vi "BUILD_install for dependencies core.vi"(6 "buildlog":path, 8 "error in":errorcluster, 9 "args":string[](array[string]), 11 "vipb path":path) -> (0 "error out":errorcluster)   [LabVIEW 2010]
uses:
  <vilib>/JKI/VIPM API/VIPM API_vipm_api.lvlib
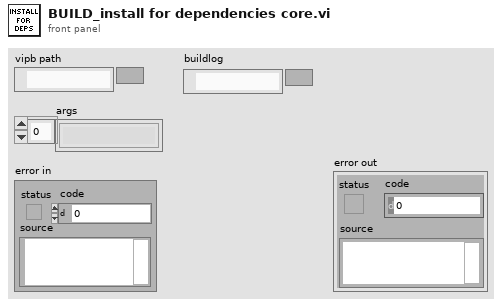
[diagram p1: front panel]
types:
  T1 = typedef "VIPM API_vipm_api.lvlib/Library Contents Cluster_vipm_api.ctl" = cluster{"Package Name":string, "Version":string, "Display Name":string, "Repository Name":string, "Company Name":string, "License Type":string, "Installed":bool, "Deprecated":bool, "Dependency or Conflict Problem":bool, "Downloaded":bool}
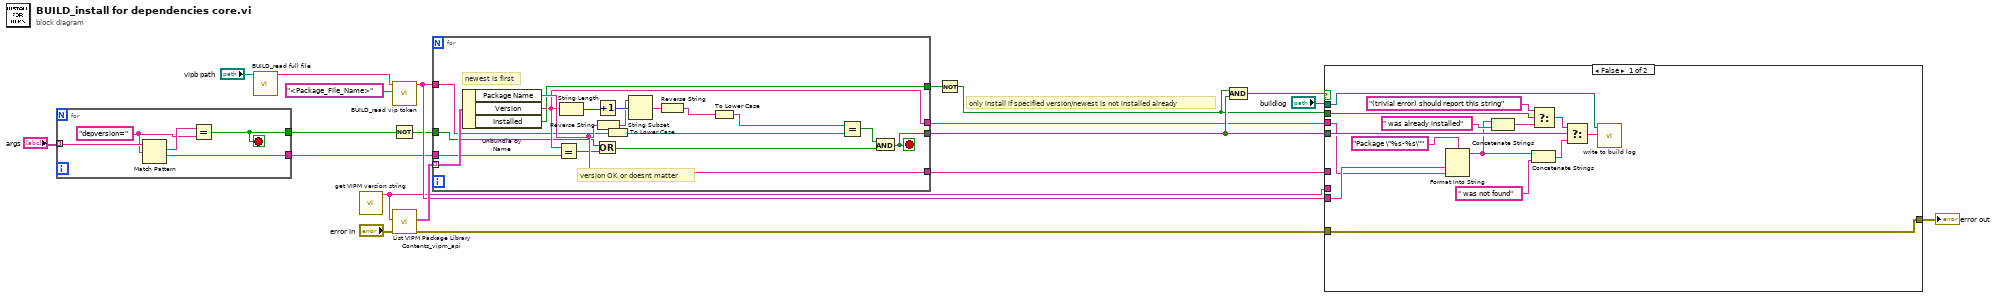
[diagram p0: block diagram]
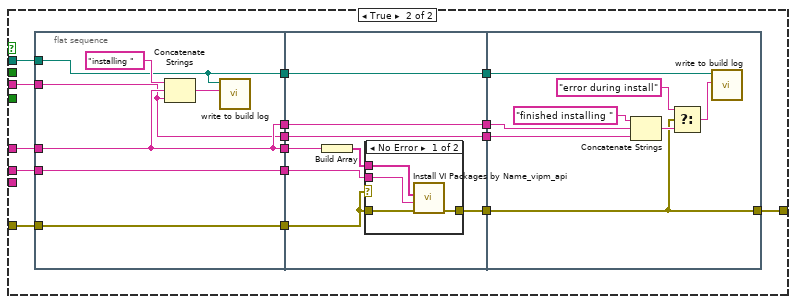
[diagram p2: hidden frame]
diagram:
  # "only install if specified version/newest is not installed already"
  n1 = for {
    tunnel: "args" -> [w25] mode=indexing
    tunnel: [w22] -> w3
    tunnel: [w21] -> w2
    stop <- w21 stop-if-true
    w23 = "depversion=" ("regular expression")
    n2 = Match Pattern(string=w25, regular expression=w23) -> (match substring=w24:string, after substring=w22:string)  [unwired: 1 in, 2 out]
    n3 = Equal?(x=w24, y=w23) -> (x = y?=w21:bool)
  }
  n4 = call "BUILD_read full file.vi"("vip file"="vipb path") -> ("data"=w19:string)  [unwired: 9 in, 1 out]
  n5 = call "get VIPM version string.vi"() -> ("version string"=w5:string)  [unwired: 11 in]
  n6 = Not(x=w2) -> (.not. x?=w1:bool)
  n7 = call "BUILD_read vip token.vi"("regular expression"="<Package_File_Name>", "data"=w19) -> ("trimmed string"=w7:string)  [unwired: 9 in]
  n8 = call <vilib>:"List VIPM Package Library Contents_vipm_api.vi"("error in (no error)"="error in", "LabVIEW Version"=w5) -> ("error out"=w17:errorcluster, "Library Contents []"=w16:T1[])  [unwired: 8 in]
  n9 = for {
    tunnel: w16 -> [w43] mode=indexing
    tunnel: [w38] -> w18
    tunnel: [w31] -> w9
    tunnel: w7 -> [w29]
    tunnel: [w36] -> w12
    tunnel: [w34] -> w4
    tunnel: w3 -> [w35]
    tunnel: w1 -> [w32]
    stop <- w31 stop-if-true
    # "version OK or doesnt matter"
    # "newest is first"
    n10 = Unbundle By Name(w43) -> ("Package Name"=w38:string, "Version"=w34:string, "Installed"=w36:bool)
    n11 = Equal?(x=w34, y=w35) -> (x = y?=w33:bool)
    n12 = String Length(string=w34) -> (length=w42:i32)
    n13 = Increment(x=w42) -> (x+1=w41:i32)
    n14 = Or(x=w32, y=w33) -> (x .or. y?=w30:bool)
    n15 = Reverse String(1:w38) -> (0:w40:string)
    n16 = To Lower Case(string=w29) -> (all lower case string=w28:string)
    n17 = String Subset(string=w40, offset (0)=w41) -> (substring=w39:string)  [unwired: 1 in]
    n18 = Reverse String(1:w39) -> (0:w27:string)
    n19 = To Lower Case(string=w27) -> (all lower case string=w26:string)
    n20 = Equal?(x=w26, y=w28) -> (x = y?=w37:bool)
    n21 = And(x=w37, y=w30) -> (x .and. y?=w31:bool)
  }
  n22 = Not(x=w12) -> (.not. x?=w8:bool)
  n23 = And(x=w8, y=w9) -> (x .and. y?=w13:bool)
  n24 = case shown="False" w13 {
    tunnel: [w58 w72] -> w14
    tunnel: w5 -> [_ w73]
    tunnel: w17 -> [w58 w71]
    tunnel: w18 -> [_ w74]
    tunnel: "buildlog" -> [w57 w66]
    tunnel: w9 -> [w56 _]
    tunnel: w8 -> [w51 _]
    tunnel: w7 -> [w55 _]
    tunnel: w4 -> [w44 w61]
    frame False {
      n25 = Format Into String(format string="Package \"%s-%s\"", w55, w44) -> (resulting string=w48:string)  [unwired: 2 in, 1 out]
      n26 = Concatenate Strings(w48, " was already installed" ("string")) -> (w47:string)
      n27 = Select(t="(trivial error) should report this string", s=w51, f=w47) -> (s? t:f=w46:string)
      n28 = Concatenate Strings(w48, " was not found" ("string")) -> (w53:string)
      n29 = Select(t=w46, s=w56, f=w53) -> (s? t:f=w50:string)
      n30 = call "write to build log.vi"("text"=w50, "log"=w57) -> ()  [unwired: 10 in]
    }
    frame True {
      n31 = flat-sequence {
        tunnel: w71 -> [w80]
        tunnel: w73 -> [w81]
        tunnel: w74 -> [w76]
        tunnel: [w76] -> w69
        tunnel: [w81] -> w68
        tunnel: [w80] -> w67
        tunnel: w66 -> [w77]
        tunnel: [w77] -> w64
        tunnel: [w76] -> w63
        tunnel: w61 -> [w75]
        tunnel: [w75] -> w60
        tunnel: [w86] -> w70
        tunnel: w69 -> [w89]
        tunnel: w68 -> [w87]
        tunnel: w67 -> [w85]
        tunnel: [w84] -> w65
        tunnel: w64 -> [w84]
        tunnel: w63 -> [w83]
        tunnel: [w83] -> w62
        tunnel: w60 -> [w82]
        tunnel: [w82] -> w59
        tunnel: [w97] -> w72
        tunnel: w70 -> [w97]
        tunnel: w65 -> [w101]
        tunnel: w62 -> [w100]
        tunnel: w59 -> [w95]
        frame #0 {
          n32 = Concatenate Strings("installing " ("string"), w76, w75) -> (w78:string)
          n33 = call "write to build log.vi"("text"=w78, "log"=w77) -> ()  [unwired: 10 in]
        }
        frame #1 {
          n34 = Build Array(w89) -> (w88:string[])
          n35 = case shown="No Error" w85 {
            tunnel: w88 -> [w93 _]
            tunnel: w87 -> [w92 _]
            tunnel: w85 -> [w91 w94]
            tunnel: [w90 w94] -> w86
            frame No Error {
              n36 = call <vilib>:"Install VI Packages by Name_vipm_api.vi"("error in (no error)"=w91, "LabVIEW Version"=w92, "Package Names to Install []"=w93) -> ("error out"=w90:errorcluster)  [unwired: 8 in]
            }
            frame Error {
            }
          }
        }
        frame #2 {
          n37 = Concatenate Strings("finished installing " ("string"), w100, w95) -> (w99:string)
          n38 = Select(t="error during install", s=w97, f=w99) -> (s? t:f=w98:string)
          n39 = call "write to build log.vi"("text"=w98, "log"=w101) -> ()  [unwired: 10 in]
        }
      }
    }
  }
  "error out" <- w14
